vi "set RBW or VBW.vi"(6 "BW Auto?":bool, 8 "error in (no error)":errorcluster, 9 "BW Type":T1, 10 "BW Value (Hz)":dbl format="%#_6p", 11 "Keysight 9020A in":refnum<class "Keysight 9020A.lvclass">) -> (0 "error out":errorcluster, 3 "Keysight 9020A out":refnum<class "Keysight 9020A.lvclass">)   [LabVIEW 2023, in "Spectrum Analyzer.lvlib" / "Keysight 9020A.lvclass"]
doc: "[RBW Setting]\n* For FSV-40\nParameters:\n<Bandwidth> refer to data sheet\n *RST: (AUTO is set to ON)\nExample:\n BAND 1 MHz\n Sets the resolution bandwidth to 1 MHz\n\n[VBW Setting]\n* For FSV-40\nParameters:\n<Bandwidth> refer to data sheet\n*RST: (AUTO is set to ON)\nExample: BAND:VID 10 kHz"
uses:
  Keysight 9020A.lvclass
  TYPE DEFINITION/TYPE RBW and VBW Select.ctl
  Keysight 9020A.lvclass/Keysight 9020A.ctl
  Spectrum Analyzer.lvlib
  <vilib>/ErrorRing/Error Ring.xnode
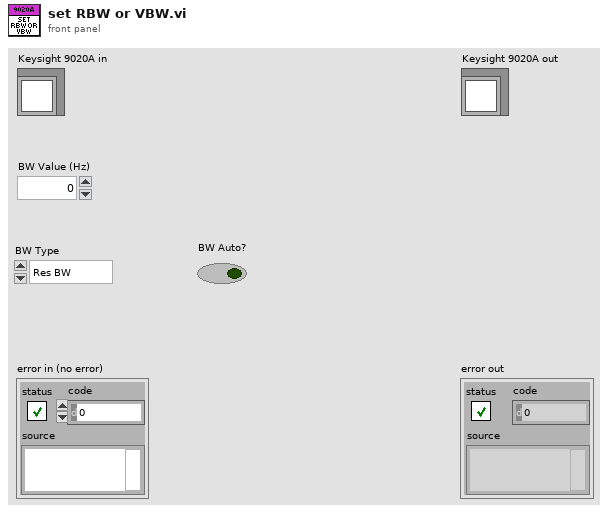
[diagram p1: front panel]
types:
  T1 = typedef "Spectrum Analyzer.lvlib/TYPE RBW and VBW Select.ctl" = enum16{"Res BW", "Video BW"}
  T2 = typedef "Spectrum Analyzer.lvlib/TYPE Measurement Preset.ctl" = enum16{"Sweep SA Mode", "Channel Power", "Occupied BW", "ACP", "Spurious Emission", "Spurious Emission Mask", "Burst Power (Transmit Power)"}
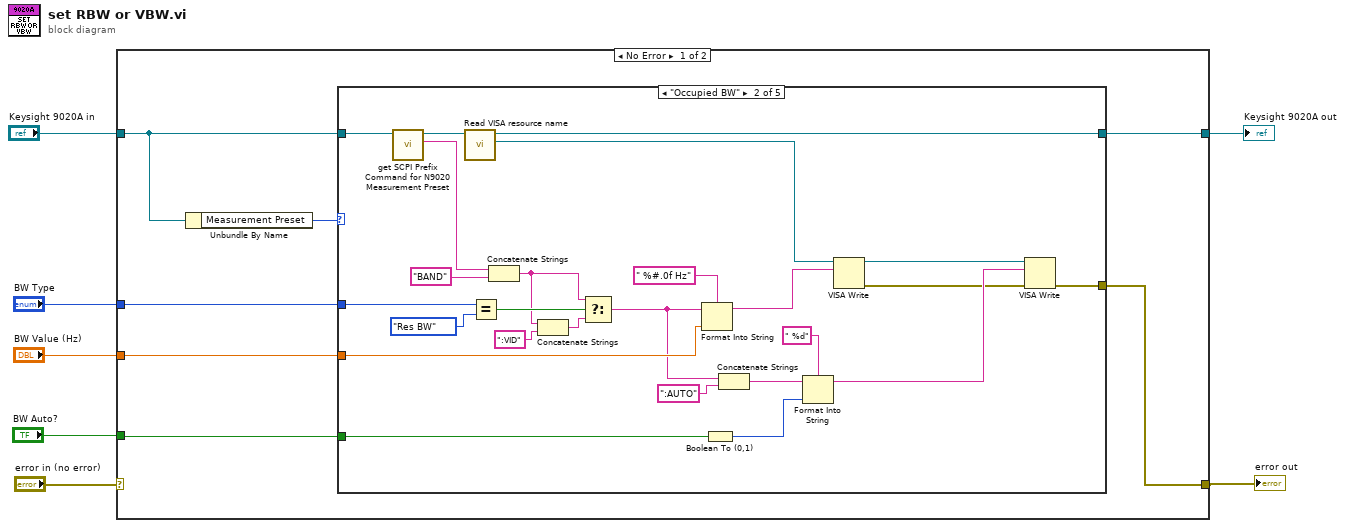
[diagram p0: block diagram]
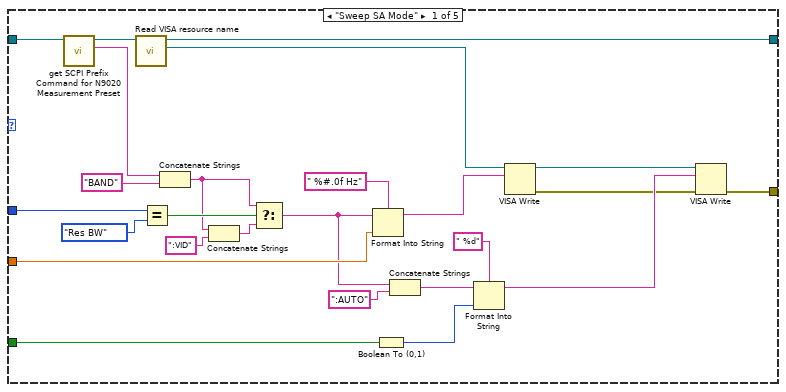
[diagram p2: hidden frame]
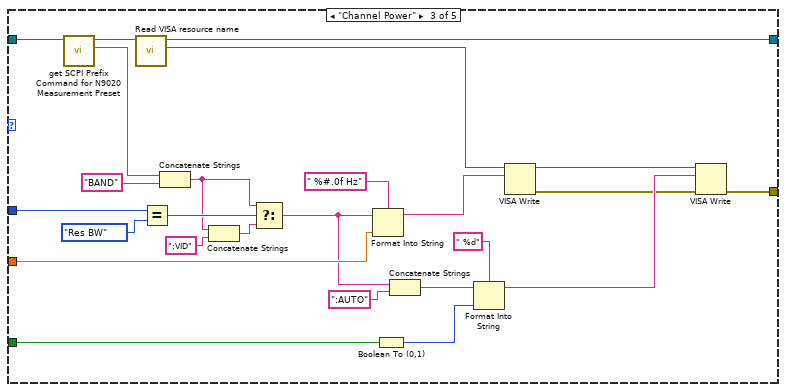
[diagram p3: hidden frame]
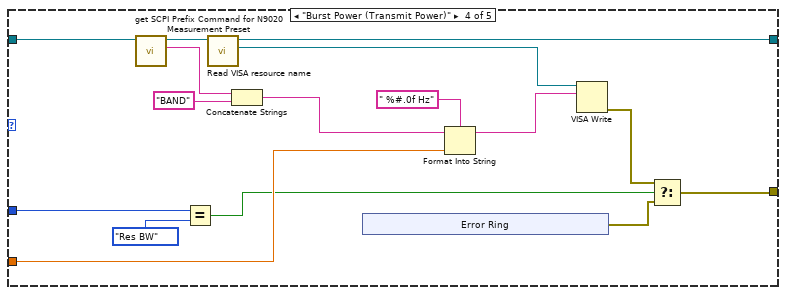
[diagram p4: hidden frame]
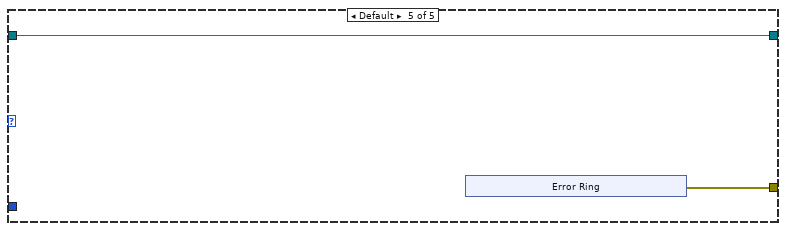
[diagram p5: hidden frame]
diagram:
  n1 = case shown="No Error" "error in (no error)" {
    selector: "error in (no error)" -> [_ w110]
    tunnel: "Keysight 9020A in" -> [w9 w111]
    tunnel: [w14 w111] -> w6
    tunnel: [w13 w110] -> w4
    tunnel: "BW Auto?" -> [w10 _]
    tunnel: "BW Value (Hz)" -> [w11 _]
    tunnel: "BW Type" -> [w12 _]
    frame No Error {
      n2 = Unbundle By Name(w9) -> ("Measurement Preset"=w8:T2)
      n3 = case shown="\"Occupied BW\"" w8 {
        tunnel: [w39 w64 w89 w97 w108] -> w14
        tunnel: [w31 w56 w81 w90 w107] -> w13
        tunnel: w12 -> [w30 w55 w80 w95 _]
        tunnel: w11 -> [w27 w52 w77 w96 _]
        tunnel: w10 -> [w23 w48 w73 _ _]
        tunnel: w9 -> [w15 w40 w65 w98 w108]
        frame "Sweep SA Mode" {
          n4 = call "get SCPI Prefix Command for N9020 Measurement Preset.vi"("Keysight 9020A in"=w15) -> ("SCPI Prefix Command"=w20:string, "Keysight 9020A out"=w21:refnum<class "Keysight 9020A.lvclass">)  [unwired: 8 in, 1 out]
          n5 = call "Read VISA resource name.vi"("Keysight 9020A in"=w21) -> ("VISA resource name"=w38:refnum<visa-resource-name>, "Keysight 9020A out"=w39:refnum<class "Keysight 9020A.lvclass">)  [unwired: 8 in, 1 out]
          n6 = Equal?(x=w30, y=TYPE_RBW_and_VBW_Select."Res BW") -> (x = y?=w28:bool)
          n7 = Concatenate Strings(w20, "BAND") -> (w18:string)
          n8 = Concatenate Strings(w18, ":VID") -> (w16:string)
          n9 = Select(t=w18, s=w28, f=w16) -> (s? t:f=w26:string)
          n10 = Format Into String(format string=" %#.0f Hz", initial string=w26, w27) -> (resulting string=w37:string)  [unwired: 1 in, 1 out]
          n11 = Boolean To (0,1)(Boolean=w23) -> (0, 1=w22:i16)
          n12 = Concatenate Strings(w26, ":AUTO" ("string")) -> (w24:string)
          n13 = Format Into String(format string=" %d", initial string=w24, w22) -> (resulting string=w34:string)  [unwired: 1 in, 1 out]
          n14 = VISA Write(VISA resource name=w38, write buffer=w37) -> (VISA resource name out=w33:refnum<visa-resource-name>, error out=w32:errorcluster)  [unwired: 1 in, 1 out]
          n15 = VISA Write(VISA resource name=w33, write buffer=w34, error in (no error)=w32) -> (error out=w31:errorcluster)  [unwired: 2 out]
        }
        frame "Occupied BW" {
          n16 = call "get SCPI Prefix Command for N9020 Measurement Preset.vi"("Keysight 9020A in"=w40) -> ("SCPI Prefix Command"=w45:string, "Keysight 9020A out"=w46:refnum<class "Keysight 9020A.lvclass">)  [unwired: 8 in, 1 out]
          n17 = call "Read VISA resource name.vi"("Keysight 9020A in"=w46) -> ("VISA resource name"=w63:refnum<visa-resource-name>, "Keysight 9020A out"=w64:refnum<class "Keysight 9020A.lvclass">)  [unwired: 8 in, 1 out]
          n18 = Equal?(x=w55, y=TYPE_RBW_and_VBW_Select."Res BW") -> (x = y?=w53:bool)
          n19 = Concatenate Strings(w45, "BAND") -> (w43:string)
          n20 = Concatenate Strings(w43, ":VID") -> (w41:string)
          n21 = Select(t=w43, s=w53, f=w41) -> (s? t:f=w51:string)
          n22 = Format Into String(format string=" %#.0f Hz", initial string=w51, w52) -> (resulting string=w62:string)  [unwired: 1 in, 1 out]
          n23 = Boolean To (0,1)(Boolean=w48) -> (0, 1=w47:i16)
          n24 = Concatenate Strings(w51, ":AUTO" ("string")) -> (w49:string)
          n25 = Format Into String(format string=" %d", initial string=w49, w47) -> (resulting string=w59:string)  [unwired: 1 in, 1 out]
          n26 = VISA Write(VISA resource name=w63, write buffer=w62) -> (VISA resource name out=w58:refnum<visa-resource-name>, error out=w57:errorcluster)  [unwired: 1 in, 1 out]
          n27 = VISA Write(VISA resource name=w58, write buffer=w59, error in (no error)=w57) -> (error out=w56:errorcluster)  [unwired: 2 out]
        }
        frame "Channel Power" {
          n28 = call "get SCPI Prefix Command for N9020 Measurement Preset.vi"("Keysight 9020A in"=w65) -> ("SCPI Prefix Command"=w70:string, "Keysight 9020A out"=w71:refnum<class "Keysight 9020A.lvclass">)  [unwired: 8 in, 1 out]
          n29 = call "Read VISA resource name.vi"("Keysight 9020A in"=w71) -> ("VISA resource name"=w88:refnum<visa-resource-name>, "Keysight 9020A out"=w89:refnum<class "Keysight 9020A.lvclass">)  [unwired: 8 in, 1 out]
          n30 = Equal?(x=w80, y=TYPE_RBW_and_VBW_Select."Res BW") -> (x = y?=w78:bool)
          n31 = Concatenate Strings(w70, "BAND") -> (w68:string)
          n32 = Concatenate Strings(w68, ":VID") -> (w66:string)
          n33 = Select(t=w68, s=w78, f=w66) -> (s? t:f=w76:string)
          n34 = Format Into String(format string=" %#.0f Hz", initial string=w76, w77) -> (resulting string=w87:string)  [unwired: 1 in, 1 out]
          n35 = Boolean To (0,1)(Boolean=w73) -> (0, 1=w72:i16)
          n36 = Concatenate Strings(w76, ":AUTO" ("string")) -> (w74:string)
          n37 = Format Into String(format string=" %d", initial string=w74, w72) -> (resulting string=w84:string)  [unwired: 1 in, 1 out]
          n38 = VISA Write(VISA resource name=w88, write buffer=w87) -> (VISA resource name out=w83:refnum<visa-resource-name>, error out=w82:errorcluster)  [unwired: 1 in, 1 out]
          n39 = VISA Write(VISA resource name=w83, write buffer=w84, error in (no error)=w82) -> (error out=w81:errorcluster)  [unwired: 2 out]
        }
        frame "Burst Power (Transmit Power)" {
          n40 = call "get SCPI Prefix Command for N9020 Measurement Preset.vi"("Keysight 9020A in"=w98) -> ("SCPI Prefix Command"=w101:string, "Keysight 9020A out"=w102:refnum<class "Keysight 9020A.lvclass">)  [unwired: 8 in, 1 out]
          n41 = Equal?(x=w95, y=TYPE_RBW_and_VBW_Select."Res BW") -> (x = y?=w93:bool)
          n42 = call "Read VISA resource name.vi"("Keysight 9020A in"=w102) -> ("VISA resource name"=w105:refnum<visa-resource-name>, "Keysight 9020A out"=w97:refnum<class "Keysight 9020A.lvclass">)  [unwired: 8 in, 1 out]
          n43 = Concatenate Strings(w101, "BAND") -> (w99:string)
          n44 = xnode "Error Ring"() -> ("error out"=w91:errorcluster)
          n45 = Format Into String(format string=" %#.0f Hz", initial string=w99, w96) -> (resulting string=w104:string)  [unwired: 1 in, 1 out]
          n46 = VISA Write(VISA resource name=w105, write buffer=w104) -> (error out=w92:errorcluster)  [unwired: 1 in, 2 out]
          n47 = Select(t=w92, s=w93, f=w91) -> (s? t:f=w90:errorcluster)
        }
        frame Default {
          n48 = xnode "Error Ring"() -> ("error out"=w107:errorcluster)
        }
      }
    }
    frame Error {
    }
  }
  "error out" <- w4
  "Keysight 9020A out" <- w6
